vi "Read Modules Configurations.vi"(8 "error in":errorcluster, 11 "Engine Parent in":refnum<class "Engine Parent Editor Node.lvclass">) -> (0 "error out":errorcluster, 2 "Component Configurations":refnum<class "TBM module configuration.lvclass">[](array[class]), 3 "Engine Parent out":refnum<class "Engine Parent Editor Node.lvclass">)   [LabVIEW 2013, in "PL Framework Configuration Tool.lvlib" / "Engine Parent Editor Node.lvclass"]
uses:
  Engine Parent Editor Node.lvclass
  <vilib>/NI/Tag Bus Module Framework/module configuration/TBM module configuration.lvclass
  <vilib>/NI/Configuration Framework/Node/NISE_CEF_Node.lvclass/NISE_CEF_Node.ctl
  Module editor node/module editor node.lvclass
  <vilib>/NI/Configuration Framework/Node/ReadChildren.vi
  <vilib>/NI/Configuration Framework/Node/NISE_CEF_Node.lvclass
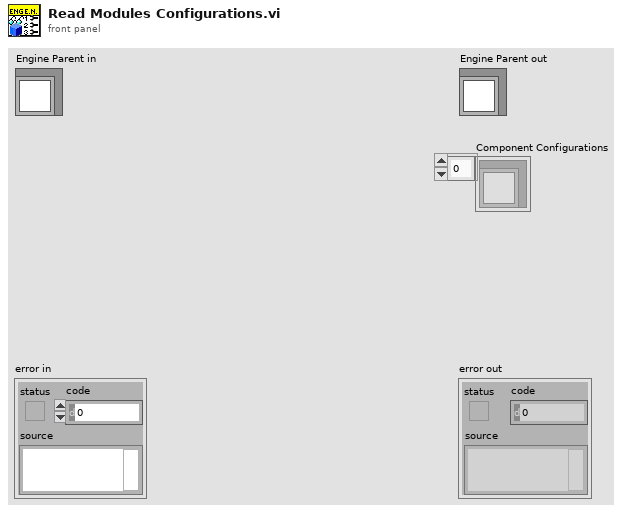
[diagram p1: front panel]
types:
  T1 = typedef "NISE_CEF_Node.lvclass/NodeRef.ctl" = refnum<data-value>
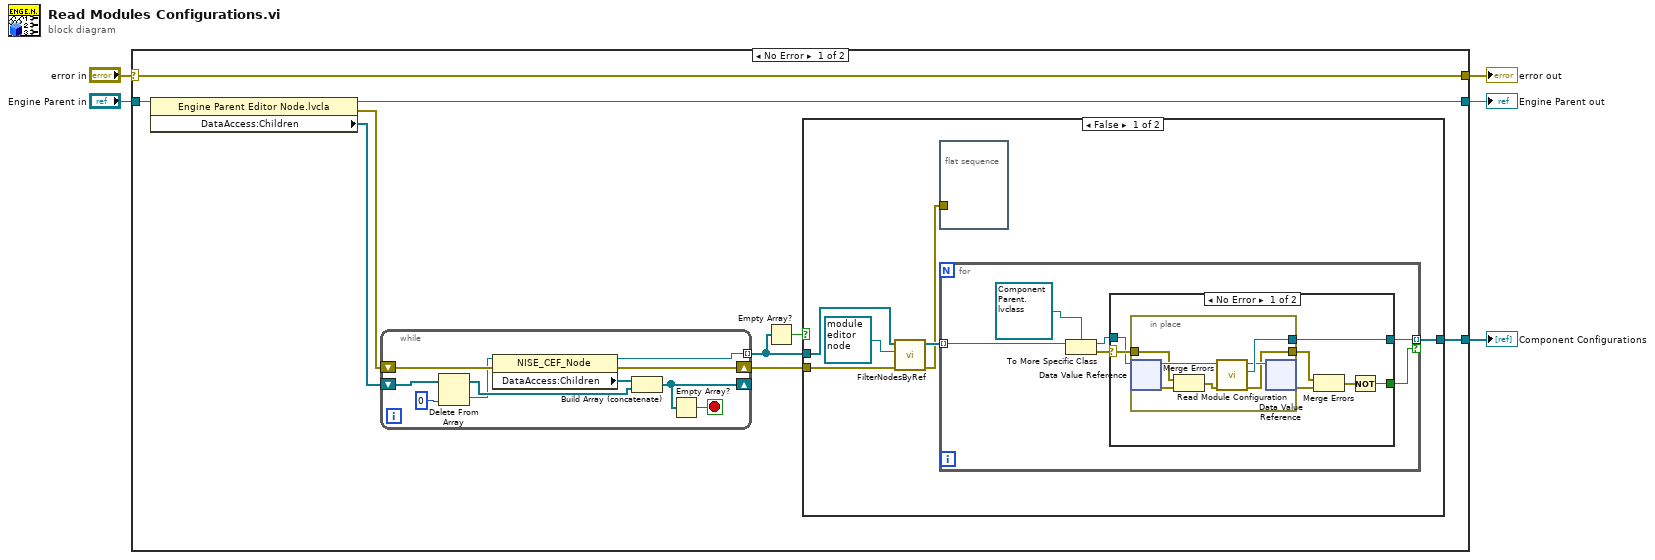
[diagram p0: block diagram]
diagram:
  n1 = case shown="No Error" "error in" {
    selector: "error in" -> [w14 w51]
    tunnel: [w14 w51] -> w4
    tunnel: [w8 w52] -> w2
    tunnel: "Engine Parent in" -> [w9 w52]
    tunnel: [w12 _] -> w1
    frame No Error {
      n2 = property class="Engine Parent Editor Node.lvcla"(reference=w9) -> (reference out=w8:refnum<class "Engine Parent Editor Node.lvclass">, error out=w10:errorcluster, "DataAccess:Children"=w11:T1[])  [unwired: 1 in]
      n3 = while {
        shift-right: [w17] -> _
        shift-left: w11 -> [w24]
        shift-right: [w21] -> w7
        shift-left: w10 -> [w22]
        tunnel: [w15] -> w6 mode=indexing
        stop <- w16 stop-if-true
        n4 = Delete From Array(array=w24, index=0) -> (deleted portion=w19:T1, array with subset deleted=w20:T1[])  [unwired: 1 in]
        n5 = property class="NISE_CEF_Node"(reference=w19, error in=w22) -> (reference out=w15:T1, error out=w21:errorcluster, "DataAccess:Children"=w18:T1[])
        n6 = Build Array (concatenate)(w18, w20) -> (w17:T1[])
        n7 = Empty Array?(array=w17) -> (empty?=w16:bool)
      }
      n8 = Empty Array?(array=w6) -> (empty?=w13:bool)
      n9 = case shown="False" w13 {
        tunnel: [w30 _] -> w12
        tunnel: w7 -> [w26 _]
        tunnel: w6 -> [w25 _]
        frame False {
          n10 = call <vilib>:"FilterNodesByRef.vi"("error in"=w26, "NISE_CEF_Node"=refnum<class "module editor node.lvclass"> refnum ("Component Parent.lvclass"), "nodes"=w25) -> ("error out"=w27:errorcluster, "filtered nodes"=w29:refnum<data-value>[])  [unwired: 7 in]
          n11 = flat-sequence {
            tunnel: w27 -> [_]
            frame #0 {
            }
          }
          n12 = for {
            tunnel: w29 -> [w36] mode=indexing
            tunnel: [w33] -> w30 mode=indexing if=w31
            n13 = To More Specific Class(target class=refnum<data-value> refnum ("data value reference"), reference=w36) -> (specific class reference=w34:refnum<data-value>, error out=w32:errorcluster)  [unwired: 1 in]
            n14 = case shown="No Error" w32 {
              selector: w32 -> [w41 _]
              tunnel: w34 -> [w40 _]
              tunnel: [w39 _] -> w33
              tunnel: [w37 _] -> w31
              frame No Error {
                n15 = in-place {
                  in-place-border: [w44] -> w42
                  in-place-border: [w49] -> w39
                  in-place-border: w41 -> [w46]
                  n16 = in-place-dvr #1(w40) -> (w50:refnum<class "module editor node.lvclass">, w47:errorcluster)
                  n17 = Merge Errors(w46, w47) -> (w45:errorcluster)
                  n18 = call "Read Module Configuration.vi"("error in"=w45, "Module Editor Node in"=w50) -> ("error out"=w44:errorcluster, "module configuration"=w49:refnum<class "TBM module configuration.lvclass">, "Module Editor Node out"=w48:refnum<class "module editor node.lvclass">)  [unwired: 7 in]
                  n19 = in-place-dvr #1(w48) -> (w43:errorcluster)  [unwired: 1 out]
                }
                n20 = Merge Errors(w42, w43) -> (w38:errorcluster)
                n21 = Not(x=w38) -> (.not. x?=w37:bool)
              }
              frame Error {
              }
            }
          }
        }
        frame True {
        }
      }
    }
    frame Error {
    }
  }
  "error out" <- w4
  "Engine Parent out" <- w2
  "Component Configurations" <- w1
